vi "TagDB Read Data Example.vi"() -> ()   [LabVIEW 2017]
uses:
  TagDB Application Example/DEF-SineSettings.ctl
  c988338c-dfcd-45ae-a170-0c12240f6647.vi
  6f91cf01-4a07-448c-baa5-5edfb62a1f80.vi
  0c6764e1-d24c-46ec-b904-80df9fc25c48.vi
  311d1dde-ba83-4290-9989-c19af25e0215.vi
  417c3fab-24f5-4ead-bd8e-e5dee33f60b4.vi
  0e353b74-2312-4321-b271-8cb97eec5687.vi
  7ee0633d-b234-47fd-a8cb-c9b47058b454.vi
  be7339b4-0250-4f30-a4a0-4151679fc0aa.vi
  daef70ba-cfd8-4b37-9936-87932a00d994.vi
  TagDB/_Support/DataAccess/data-Write.vi
  TagDB/_Support/URL/TRIM-BOTH-SPACE.vi
  TagDB/_Support/Error/_[error50000]Invalid DB REF.vi
  TagDB/_Support/DataAccess/TagDB Ref to DVR.vi
  TagDB/_Support/DataAccess/_NameCacher.vi
  TagDB/_Support/Error/_[error50002]Invalid DataType.vi
  TagDB/_Support/DataAccess/_datatypeChecker.vi
  <vilib>/Utility/Data Type/Get Type Information.vi
  TagDB/_Support/Error/_Build Error Cluster.vi
  TagDB/TagDB.lvlib
panel:
  out "Time Stamp 5":timestamp
  out "Value 5":dbl
  out "Time Stamp 4":timestamp
  out "Value 4":dbl
  out "Value 3":cluster{"1":dbl, "2":dbl}
  out "Time Stamp 3":timestamp
  out "Time Stamp 2":timestamp
  out "Time Stamp":timestamp
  out "Value 2":T1
  out "Value":T2
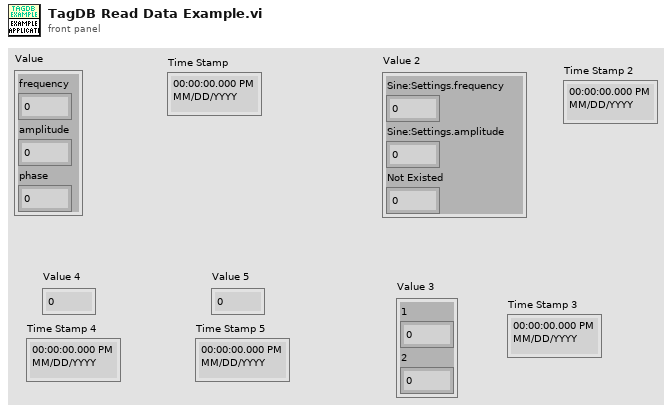
[diagram p1: front panel]
types:
  T1 = cluster{"Sine:Settings.frequency":dbl, "Sine:Settings.amplitude":dbl, "Not Existed":dbl}
  T2 = cluster{"frequency":dbl, "amplitude":dbl, "phase":dbl}
  T3 = typedef "DEF-SineSettings.ctl" = cluster{"frequency":dbl, "amplitude":dbl, "phase":dbl, "sampling info":cluster{"Fs":dbl, "#s":dbl}}
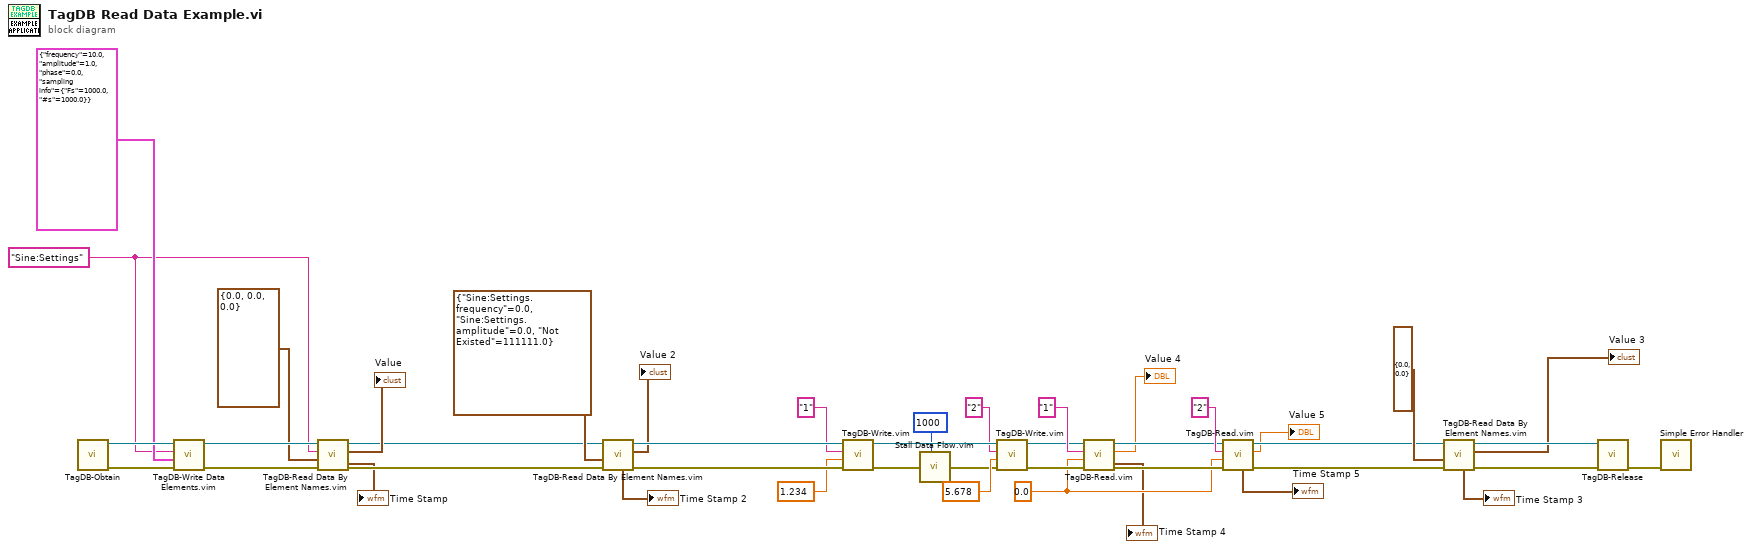
[diagram p0: block diagram]
diagram:
  w5 = 0.0
  w37 = "Sine:Settings" ("name")
  n1 = call "TagDB-Obtain.vi"() -> ("error out"=w41:errorcluster, "TagDB"=w42:refnum<k1>)  [unwired: 5 in, 1 out]
  n2 = call "TagDB-Write Data Elements.vim"("error in (no error)"=w41, "Value"=T3 {"frequency"=10.0, "amplitude"=1.0, "phase"=0.0, "sampling info"={"Fs"=1000.0, "#s"=1000.0}} ("Sine Settings"), "root tag"=w37, "TagDB"=w42) -> ("error out"=w39:errorcluster, "TagDB(dup)"=w38:refnum<k1>)  [unwired: 5 in, 1 out]
  n3 = call "TagDB-Read Data By Element Names.vim"("error in (no error)"=w39, "Type(empty to read as variant)"=T2 {"frequency"=0.0, "amplitude"=0.0, "phase"=0.0} ("Sine Settings"), "Root Tag"=w37, "TagDB"=w38) -> ("error out"=w32:errorcluster, "Value"=→"Value":T2, "TagDB(dup)"=w33:refnum<k1>, "Time Stamp"=→"Time Stamp":timestamp)  [unwired: 4 in]
  n4 = call "TagDB-Read Data By Element Names.vim"("error in (no error)"=w32, "Type(empty to read as variant)"=T1 {"Sine:Settings.frequency"=0.0, "Sine:Settings.amplitude"=0.0, "Not Existed"=111111.0} ("Sine Settings"), "TagDB"=w33) -> ("error out"=w25:errorcluster, "Value"=→"Value 2":T1, "TagDB(dup)"=w31:refnum<k1>, "Time Stamp"=→"Time Stamp 2":timestamp)  [unwired: 5 in]
  n5 = call "TagDB-Write.vim"("error in (no error)"=w25, "Value"=1.234, "tag"="1", "TagDB"=w31) -> ("error out"=w24:errorcluster, "TagDB(dup)"=w27:refnum<k1>)  [unwired: 5 in, 1 out]
  n6 = call "Stall Data Flow.vim"("value in"=w24, "milliseconds to wait"=u32 1000) -> ("value out"=w18:errorcluster)  [unwired: 1 out]
  n7 = call "TagDB-Write.vim"("error in (no error)"=w18, "Value"=5.678, "tag"="2", "TagDB"=w27) -> ("error out"=w8:errorcluster, "TagDB(dup)"=w9:refnum<k1>)  [unwired: 5 in, 1 out]
  n8 = call "TagDB-Read.vim"("error in (no error)"=w8, "Type(empty to read as variant)"=w5, "name"="1" ("tag"), "TagDB"=w9) -> ("error out"=w11:errorcluster, "Value"=→"Value 4":dbl, "TagDB(dup)"=w10:refnum<k1>, "Time Stamp"=→"Time Stamp 4":timestamp)  [unwired: 2 in, 2 out]
  n9 = call "TagDB-Read.vim"("error in (no error)"=w11, "Type(empty to read as variant)"=w5, "name"="2" ("tag"), "TagDB"=w10) -> ("error out"=w6:errorcluster, "Value"=→"Value 5":dbl, "TagDB(dup)"=w7:refnum<k1>, "Time Stamp"=→"Time Stamp 5":timestamp)  [unwired: 2 in, 2 out]
  n10 = call "TagDB-Read Data By Element Names.vim"("error in (no error)"=w6, "Type(empty to read as variant)"=cluster{"1":dbl, "2":dbl} {"1"=0.0, "2"=0.0} ("Sine Settings"), "TagDB"=w7) -> ("error out"=w23:errorcluster, "Value"=→"Value 3":cluster{"1":dbl, "2":dbl}, "TagDB(dup)"=w26:refnum<k1>, "Time Stamp"=→"Time Stamp 3":timestamp)  [unwired: 5 in]
  n11 = call "TagDB-Release.vi"("error in (no error)"=w23, "TagDB"=w26) -> ("error out"=w43:errorcluster)  [unwired: 9 in]
  n12 = call <vilib>:"Simple Error Handler.vi"("error in (no error)"=w43) -> ()  [unwired: 4 in, 5 out]
